vi "Arg2States.vi"(9 "Arguments":string, 10 "State":string[](array[string])) -> (2 "States Out":string)   [LabVIEW 2017]
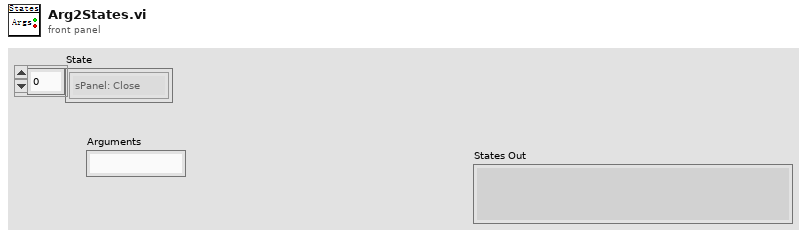
[diagram p1: front panel]
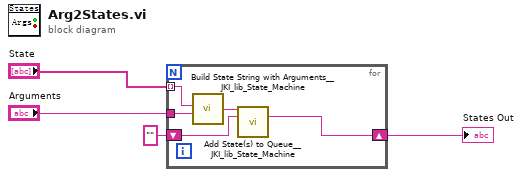
[diagram p0: block diagram]
diagram:
  n1 = for {
    tunnel: "Arguments" -> [w7]
    tunnel: "State" -> [w8] mode=indexing
    shift-right: [w6] -> w2
    shift-left: "" ("States Out") -> [w5]
    n2 = call <vilib>:"Build State String with Arguments__JKI_lib_State_Machine.vi"("Arguments (\"\")"=w7, "State"=w8) -> ("State with Arguments"=w9:string)  [unwired: 4 in]
    n3 = call <vilib>:"Add State(s) to Queue__JKI_lib_State_Machine.vi"("State(s) in Front (\"\")"=w9, "State(s) in (\"\")"=w5) -> ("States Out"=w6:string)  [unwired: 13 in]
  }
  "States Out" <- w2
